vi "Periodic Tasks.vi"(8 "error in":errorcluster) -> ()   [LabVIEW 2019]
doc: "This VI runs in parallel to other tasks. It can contain as many user-defined periodic loops as you need. These can carry out PID or other sorts of timed response."
uses:
  <vilib>/Rock Robotics/WPI/ThirdParty/JAS_Junk/TrajLib/MathUtil_Clamp.vi
  Robot Global Data.vi
  <vilib>/Rock Robotics/Network Tables/NT Write Number.vi
  <vilib>/Rock Robotics/WPI/ThirdParty/JAS_Junk/TrajLib/Trajectory_Library.lvlib
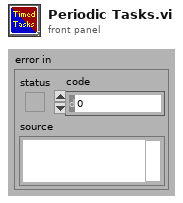
[diagram p1: front panel]
types:
  T1 = typedef "WPI_GyroDevRef.ctl" = cluster{"DevStatus":errorcluster, "Analog Channel":T2, "Gain (VoltsPerDegree/Second)":dbl, "Gyro Type":enum16{"Analog", "XRS450"}, "Handle":i32, "SPI Bus":T3, "Device Found":bool, "Sample Rate":dbl, "Calibrate On Open":bool, "Offset":dbl}
  T2 = typedef "FPGA_AIChannel.ctl" = enum8{"AI 0", "AI 1", "AI 2", "AI 3", "AI MXP 0", "AI MXP 1", "AI MXP 2", "AI MXP 3", "Invalid"}
  T3 = typedef "spi_bus.ctl" = enum16{"SPI On-Board, CS0", "SPI On-Board, CS1", "SPI On-Board, CS2", "SPI On-Board, CS3", "SPI MXP", "Invalid"}
  T4 = typedef "Trajectory_Library.lvlib/SWERVE_DRIVE_MODULE_STATE.ctl" = cluster{"Speed":dbl, "Angle":T5}
  T5 = typedef "Trajectory_Library.lvlib/ROTATION2D.ctl" = cluster{"VALUE":dbl, "COS":dbl, "SIN":dbl}
  T6 = typedef "SWERVE_DRIVE_MODULE_TYPDEF.ctl" = cluster{"SwervDriveMotor":T7, "SwerveSwerveMotor":T7, "SwerveDriveEnc":T12, "SwerveSwerveEnc":T12}
  T7 = typedef "WPI_MotorControlDeviceRef.ctl" = cluster{"DeviceStatus":errorcluster, "Type":T8, "PWM":cluster{"PWM Channel":T9, "DeadBand":T10}, "CAN":cluster{"Device Number":u8, "SetOutput VI Ref":variant, "GetOutput VI Ref":variant, "Enable VI Ref":variant, "Disable VI Ref":variant, "Data":variant}, "Invert":bool, "DIO PWM":cluster{"PWM \"Enable\" Channel":T9, "DIOChannel":T11, "PWM Rate":dbl}}
  T8 = typedef "WPI_MotorControlType.ctl" = enum16{"PWM", "CAN", "DIO PWM"}
  T9 = typedef "FPGA_DIOPWMChannel.ctl" = enum8{"PWM 0", "PWM 1", "PWM 2", "PWM 3", "PWM 4", "PWM 5", "PWM 6", "PWM 7", "PWM 8", "PWM 9", "PWM MXP 0", "PWM MXP 1", "PWM MXP 2", "PWM MXP 3", "PWM MXP 4", "PWM MXP 5", "PWM MXP 6", "PWM MXP 7", "PWM MXP 8", "PWM MXP 9", "Invalid"}
  T10 = typedef "WPI_PWMDeadband.ctl" = cluster{"Name":string, "maxPositivePwm":i32, "minPositivePwm":i32, "centerPwm":i32, "maxNegativePwm":i32, "minNegativePwm":i32, "angularRange":u16}
  T11 = typedef "FPGA_DIOChannel.ctl" = enum8{"DIO 0", "DIO 1", "DIO 2", "DIO 3", "DIO 4", "DIO 5", "DIO 6", "DIO 7", "DIO 8", "DIO 9", "DIO MXP 0", "DIO MXP 1", "DIO MXP 2", "DIO MXP 3", "DIO MXP 4", "DIO MXP 5", "DIO MXP 6", "DIO MXP 7", "DIO MXP 8", "DIO MXP 9", "DIO MXP 10", "DIO MXP 11", "DIO MXP 12", "DIO MXP 13", "DIO MXP 14", "DIO MXP 15", "SPI Port CS1", "SPI Port CS2", "SPI Port CS3", "SPI Port MISO", "SPI Port MOSI", "Invalid"}
  T12 = typedef "WPI_EncoderDevRef.ctl" = cluster{"DevStatus":errorcluster, "EncoderIndex":T13, "CounterIndex":T14, "DistancePerCount":dbl, "Decoding Type":T15}
  T13 = typedef "FPGA_EncoderIdx.ctl" = enum8{"Enc 0", "Enc 1", "Enc 2", "Enc 3", "Enc 4", "Enc 5", "Enc 6", "Enc 7", "Invalid"}
  T14 = typedef "FPGA_CounterCtrSystemIndex.ctl" = enum8{"Ctr 0", "Ctr 1", "Ctr 2", "Ctr 3", "Ctr 4", "Ctr 5", "Ctr 6", "Ctr 7", "Invalid"}
  T15 = typedef "WPI_EncoderType.ctl" = enum16{"1x", "2x", "4x"}
  T16 = typedef "Trajectory_Library.lvlib/SWERVE_DRIVE_KINEMATICS.ctl" = cluster{"NumModules":i32, "InverseKinematics":T17, "ForwardKinematics":T17, "Modules":T18[], "PrevCoR":T18, "SavedModuleStates":T4[]}
  T17 = typedef "NI_Matrix.lvlib/RealMatrix.ctl" = dbl[][]
  T18 = typedef "Trajectory_Library.lvlib/TRANSLATION2D.ctl" = cluster{"X":dbl, "Y":dbl}
  T19 = typedef "Trajectory_Library.lvlib/SWERVE_DRIVE_MODULE_POSITION.ctl" = cluster{"Distance":dbl, "Angle":T5, "P":bool}
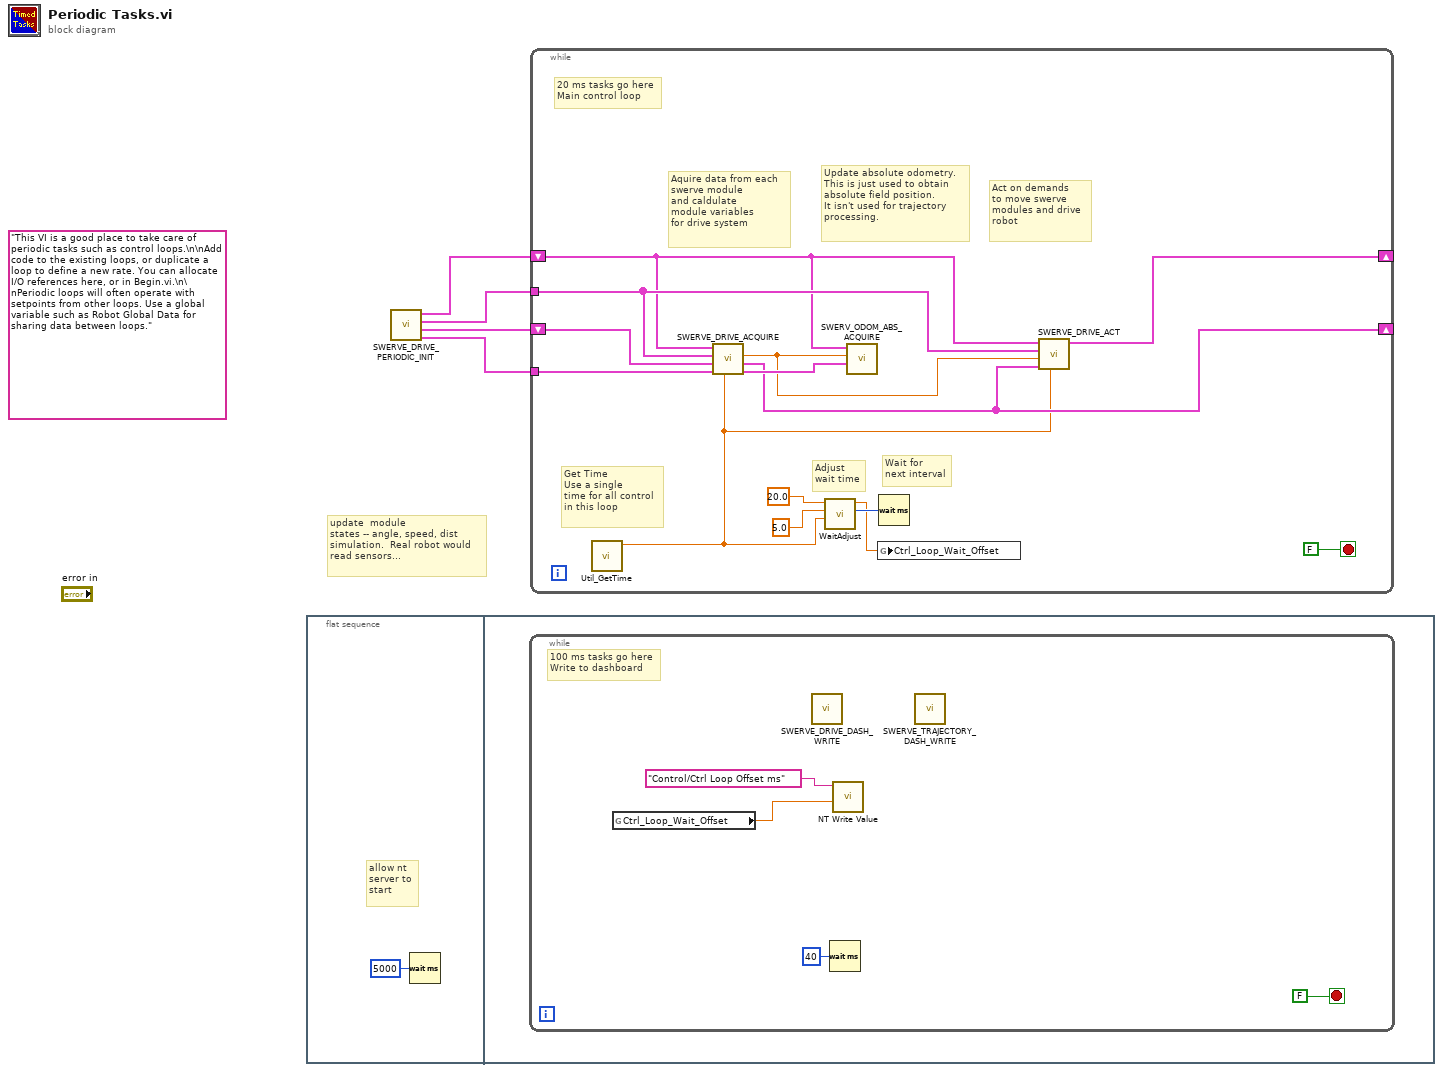
[diagram p0: block diagram]
diagram:
  (unwired) "This VI is a good place to take care of periodic tasks such as control loops.\n\nAdd code to the existing loops, or duplicate a loop to define a new rate. You can allocate I/O references here, or in Begin.vi.\n\nPeriodic loops will often operate with setpoints from other loops. Use a global variable such as Robot Global Data for sharing data between loops."
  # "update  module\nstates -- angle, speed, dist\nsimulation.  Real robot would\nread sensors..."
  n1 = flat-sequence {
    frame #0 {
      # "allow nt\nserver to \nstart"
      n2 = Wait (ms)(milliseconds to wait=u32 5000) -> ()  [unwired: 1 out]
    }
    frame #1 {
      n3 = while {
        stop <- FALSE stop-if-true
        # "100 ms tasks go here\nWrite to dashboard"
        n4 = global read "Robot Global Data.vi" "Ctrl_Loop_Wait_Offset"() -> (w6:dbl)
        n5 = call "SWERVE_DRIVE_DASH_WRITE.vi"() -> ()  [unwired: 12 in]
        n6 = Wait (ms)(milliseconds to wait=u32 40) -> ()  [unwired: 1 out]
        n7 = call-poly <vilib>:"NT Write Value.vi"("Numeric"=w6, "Name"="Control/Ctrl Loop Offset ms") -> ()  [unwired: 9 in, 1 out]
        n8 = call "SWERVE_TRAJECTORY_DASH_WRITE.vi"() -> ()  [unwired: 12 in]
      }
    }
  }
  n9 = call "SWERVE_DRIVE_PERIODIC_INIT.vi"() -> ("GyroDevRef"=w1:T1, "Swerve Module Sttes"=w4:T4[], "Swerve Device References"=w2:T6[], "WERVE_DRIVE_KINEMATICS"=w3:T16)  [unwired: 8 in]
  n10 = while {
    shift-right: [w16] -> _
    shift-left: w4 -> [w21]
    tunnel: w2 -> [w20]
    shift-right: [w22] -> _
    shift-left: w3 -> [w17]
    tunnel: w1 -> [w19]
    stop <- FALSE stop-if-true
    # "Wait for\nnext interval"
    # "Adjust\nwait time"
    # "Get Time\nUse a single\ntime for all control\nin this loop"
    # "Act on demands\nto move swerve\nmodules and drive\nrobot"
    # "Aquire data from each\nswerve module\nand caldulate\nmodule variables\nfor drive system"
    # "Update absolute odometry.\nThis is just used to obtain\nabsolute field position.\nIt isn't used for trajectory\nprocessing."
    # "20 ms tasks go here\nMain control loop"
    n11 = call <vilib>:"Util_GetTime.vi"() -> ("FPGA_Time_Seconds"=w11:dbl)  [unwired: 10 in, 1 out]
    n12 = call "SWERVE_DRIVE_ACQUIRE.vi"("Pass_Through_Time"=w11, "GyroDevRef"=w19, "in Swerve Module States"=w21, "Swerve IO Reference"=w20, "in SWERVE_DRIVE_KINEMATICS"=w17) -> ("out Swerve Module Positions"=w18:T19[], "out Swerve Module States"=w16:T4[], "Gyro_Heading_Rad"=w15:dbl)  [unwired: 4 in]
    n13 = call <vilib>:"WaitAdjust.vi"("Time_SEC"=w11, "MaxDeviation_MS"=5.0, "DesiredLoopTime_MS"=20.0) -> ("AdjustedWaitTime_MS"=w12:u32, "Offset_MS"=w10:dbl)  [unwired: 7 in]
    n14 = call "SWERV_ODOM_ABS_ACQUIRE.vi"("in Swerve Module Positions"=w18, "Gyro_Heading_Rad"=w15, "in SWERVE_DRIVE_KINEMATICS"=w17) -> ()  [unwired: 9 in]
    n15 = global write "Robot Global Data.vi" "Ctrl_Loop_Wait_Offset"(w10) -> ()
    n16 = Wait (ms)(milliseconds to wait=w12) -> ()  [unwired: 1 out]
    n17 = call "SWERVE_DRIVE_ACT.vi"("Pass_Through_Time"=w11, "in Swerve Module States"=w16, "Gyro_Heading_Rad"=w15, "Swerve Drive Device Reference"=w20, "in SWERVE_DRIVE_KINEMATICS"=w17) -> ("out SWERVE_DRIVE_KINEMATICS"=w22:T16)  [unwired: 6 in]
  }
